vi "Register gRPC Methods.vi"(8 "error in (no error)":errorcluster, 11 "gRPC service in":refnum<class "CanWriterCansub.lvclass">) -> (0 "error out":errorcluster, 3 "gRPC service out":refnum<class "CanWriterCansub.lvclass">)   [LabVIEW 2021, in "CanWriterCansub_server.lvlib" / "CanWriterCansub.lvclass"]
uses:
  CanWriterCansub.lvclass
  typeDefs/Server Internal UEs.ctl
  typeDefs/Server Internal Message.ctl
  typeDefs/Server gRPC UEs.ctl
  <vilib>/gRPC/LabVIEW gRPC Library/Server API/typeDefs/gRPCId Cluster.ctl
  <vilib>/gRPC/LabVIEW gRPC Library/Shared/grpcId.ctl
  CanWriterCansub.lvclass/CanWriterCansub.ctl
  <vilib>/gRPC/LabVIEW gRPC Library/grpc-lvsupport-release.lvlib
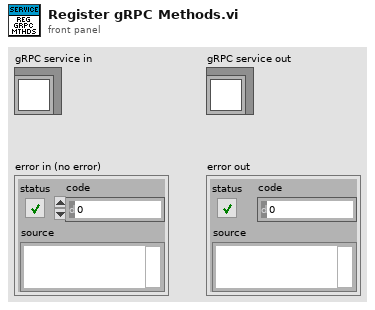
[diagram p1: front panel]
types:
  T1 = typedef "CanWriterCansub_server.lvlib/CanWriterCansub.lvclass/Server gRPC UEs.ctl" = cluster{"CanWriterCansub GetDevices gRPC UE":refnum<user-event>, "CanWriterCansub GetStatistics gRPC UE":refnum<user-event>, "CanWriterCansub SetInterfaceBlink gRPC UE":refnum<user-event>, "CanWriterCansub SendCanMessage gRPC UE":refnum<user-event>, "CanWriterCansub GetCANStatus gRPC UE":refnum<user-event>}
  T2 = typedef "CanWriterCansub_server.lvlib/CanWriterCansub.lvclass/Server Internal UEs.ctl" = cluster{"CanWriterCansub GetDevices Internal UE":refnum<user-event>, "CanWriterCansub GetStatistics Internal UE":refnum<user-event>, "CanWriterCansub SetInterfaceBlink Internal UE":refnum<user-event>, "CanWriterCansub SendCanMessage Internal UE":refnum<user-event>, "CanWriterCansub GetCANStatus Internal UE":refnum<user-event>}
  T3 = typedef "grpc-lvsupport-release.lvlib/grpcId.ctl" = u64
  T4 = typedef "CanWriterCansub_server.lvlib/CanWriterCansub.lvclass/Server Internal Message UE.ctl" = refnum<user-event>
  T5 = typedef "grpc-lvsupport-release.lvlib/gRPCId Cluster UE.ctl" = refnum<user-event>
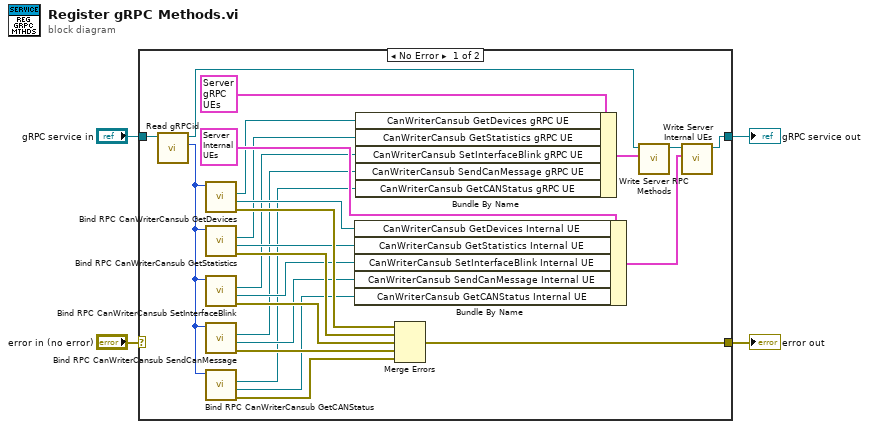
[diagram p0: block diagram]
diagram:
  n1 = case shown="No Error" "error in (no error)" {
    selector: "error in (no error)" -> [_ w30]
    tunnel: "gRPC service in" -> [w21 w31]
    tunnel: [w29 w30] -> w3
    tunnel: [w28 w31] -> w2
    frame No Error {
      n2 = call-dynamic "Read gRPCid.vi"("gRPC service in"=w21) -> ("gRPCid"=w20:T3, "gRPC service out"=w22:refnum<class "CanWriterCansub.lvclass">)  [unwired: 8 in, 1 out]
      n3 = call "Bind RPC CanWriterCansub GetDevices.vi"("gRPCid server in"=w20) -> ("error out"=w19:errorcluster, "CanWriterCansub GetDevices Internal UE"=w18:T4, "CanWriterCansub GetDevices gRPC UE"=w17:T5)  [unwired: 7 in, 1 out]
      n4 = call "Bind RPC CanWriterCansub GetStatistics.vi"("gRPCid server in"=w20) -> ("error out"=w16:errorcluster, "CanWriterCansub GetStatistics Internal UE"=w14:T4, "CanWriterCansub GetStatistics gRPC UE"=w15:T5)  [unwired: 7 in, 1 out]
      n5 = call "Bind RPC CanWriterCansub SetInterfaceBlink.vi"("gRPCid server in"=w20) -> ("error out"=w13:errorcluster, "CanWriterCansub SetInterfaceBlink Internal UE"=w12:T4, "CanWriterCansub SetInterfaceBlink gRPC UE"=w11:T5)  [unwired: 7 in, 1 out]
      n6 = call "Bind RPC CanWriterCansub SendCanMessage.vi"("gRPCid server in"=w20) -> ("error out"=w10:errorcluster, "CanWriterCansub SendCanMessage Internal UE"=w9:T4, "CanWriterCansub SendCanMessage gRPC UE"=w8:T5)  [unwired: 7 in, 1 out]
      n7 = call "Bind RPC CanWriterCansub GetCANStatus.vi"("gRPCid server in"=w20) -> ("error out"=w7:errorcluster, "CanWriterCansub GetCANStatus Internal UE"=w6:T4, "CanWriterCansub GetCANStatus gRPC UE"=w5:T5)  [unwired: 7 in, 1 out]
      n8 = Bundle By Name ("Bundle Internal UEs")(cluster=T2 {"CanWriterCansub GetDevices Internal UE"=refnum, "CanWriterCansub GetStatistics Internal UE"=refnum, "CanWriterCansub SetInterfaceBlink Internal UE"=refnum, "CanWriterCansub SendCanMessage Internal UE"=refnum, "CanWriterCansub GetCANStatus Internal UE"=refnum} ("Server Internal UEs"), "CanWriterCansub GetDevices Internal UE"=w18, "CanWriterCansub GetStatistics Internal UE"=w14, "CanWriterCansub SetInterfaceBlink Internal UE"=w12, "CanWriterCansub SendCanMessage Internal UE"=w9, "CanWriterCansub GetCANStatus Internal UE"=w6) -> (w27:T2)
      n9 = Bundle By Name ("Bundle gRPC UEs")(cluster=T1 {"CanWriterCansub GetDevices gRPC UE"=refnum, "CanWriterCansub GetStatistics gRPC UE"=refnum, "CanWriterCansub SetInterfaceBlink gRPC UE"=refnum, "CanWriterCansub SendCanMessage gRPC UE"=refnum, "CanWriterCansub GetCANStatus gRPC UE"=refnum} ("gRPC Server Method Events"), "CanWriterCansub GetDevices gRPC UE"=w17, "CanWriterCansub GetStatistics gRPC UE"=w15, "CanWriterCansub SetInterfaceBlink gRPC UE"=w11, "CanWriterCansub SendCanMessage gRPC UE"=w8, "CanWriterCansub GetCANStatus gRPC UE"=w5) -> (w24:T1)
      n10 = Merge Errors(w19, w16, w13, w10, w7) -> (w29:errorcluster)
      n11 = call "Write Server RPC Methods.vi"("Server RPC Methods"=w24, "gRPC service in"=w22) -> ("gRPC service out"=w25:refnum<class "CanWriterCansub.lvclass">)  [unwired: 8 in, 1 out]
      n12 = call "Write Server Internal UEs.vi"("Server Internal UEs"=w27, "gRPC service in"=w25) -> ("gRPC service out"=w28:refnum<class "CanWriterCansub.lvclass">)  [unwired: 8 in, 1 out]
    }
    frame Error {
    }
  }
  "error out" <- w3
  "gRPC service out" <- w2
